vi "Lab09_task1.vi"() -> ()   [LabVIEW 2022 SP3]
uses:
  <vilib>/Utility/file.llb/Write Delimited Spreadsheet (string).vi
  <vilib>/Utility/file.llb/Write Delimited Spreadsheet (DBL).vi
  <vilib>/measure/mascope.llb/Pulse Measurements N chan.vi
  <vilib>/measure/NI_MAPro.lvlib
panel:
  out "Frequency (Hz)":dbl
  out "error out":errorcluster
  out "duty cycle":dbl[](array[numeric]) format="%.2p"
  out "pulse duration":dbl[](array[numeric]) format="%.2p"
  in  "reference levels":T1={"high ref level"=90.0, "mid ref level"=50.0, "low ref level"=10.0, "ref units"=1} {"ref units" items=["absolute", "percent"]; "high ref level" format="%.2p"; "low ref level" format="%.2p"; "mid ref level" format="%.2p"}
  out "period":dbl[](array[numeric]) format="%.2p"
  in  "file path (dialog if empty)":path
  in  "number of samples":i32=5000
  out "Waveform Graph":dynamicdata(graph)
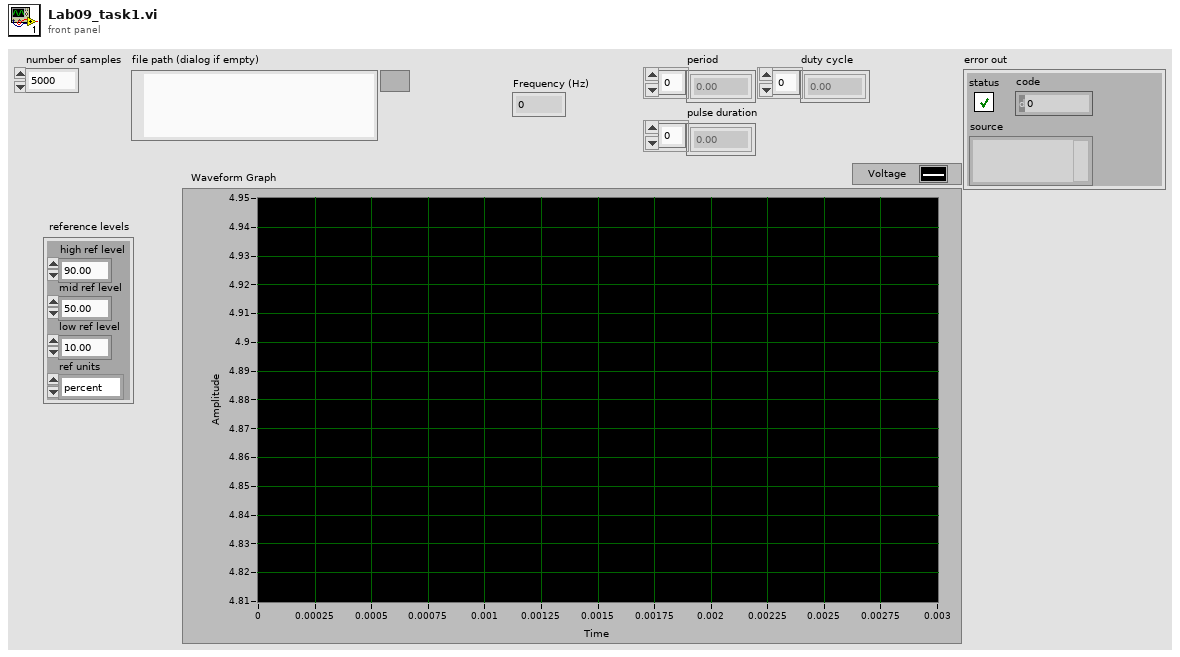
[diagram p1: front panel]
types:
  T1 = cluster{"high ref level":dbl, "mid ref level":dbl, "low ref level":dbl, "ref units":u16}
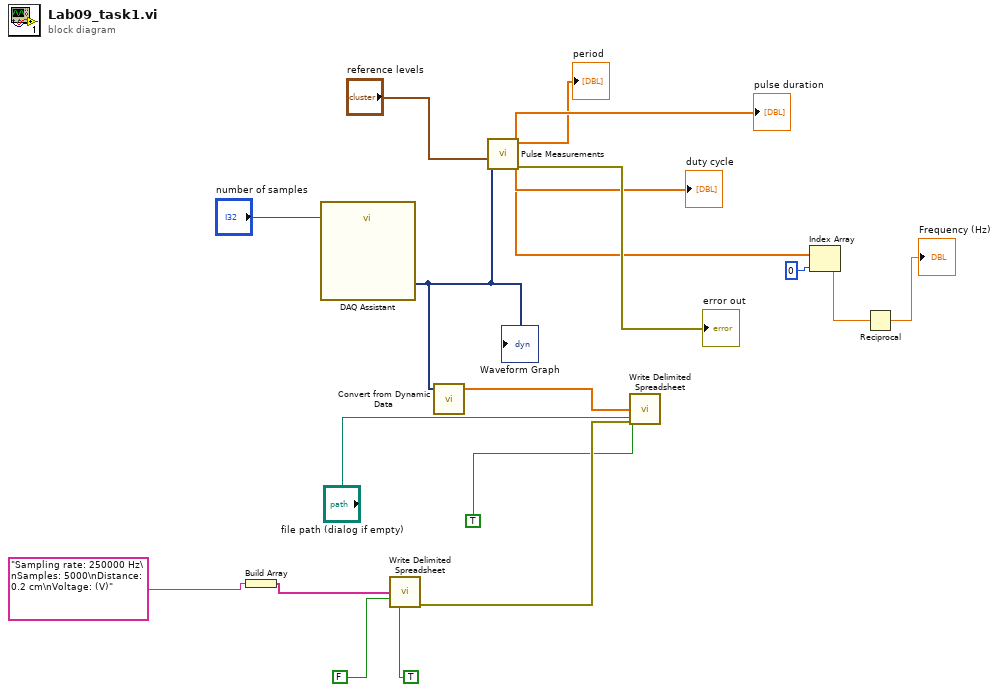
[diagram p0: block diagram]
diagram:
  n1 = Build Array("Sampling rate: 250000 Hz\nSamples: 5000\nDistance: 0.2 cm\nVoltage: (V)") -> (w16:string[])
  n2 = call "DAQ Assistant"("number of samples"="number of samples") -> ("data"=w9:dynamicdata)  [unwired: 16 in, 2 out]
  "Waveform Graph" <- w9
  n3 = call-poly <vilib>:"Write Delimited Spreadsheet.vi"("1D data"=w16, "append to file? (new file:F)"=FALSE, "transpose? (no:F)"=TRUE) -> ("error out"=w12:errorcluster)  [unwired: 11 in, 1 out]
  n4 = call "Convert from Dynamic Data"("Dynamic Data Type"=w9) -> ("Array"=w10:dbl[])  [unwired: 3 in]
  n5 = call-poly <vilib>:"Pulse Measurements.vi"("reference levels"="reference levels", "signal(s) in"=w9) -> ("error out"=→"error out":errorcluster, "duty cycle"=→"duty cycle":dbl[], "pulse duration"=→"pulse duration":dbl[], "period"=w1:dbl[])  [unwired: 5 in, 1 out]
  "period" <- w1
  n6 = call-poly <vilib>:"Write Delimited Spreadsheet.vi"("file path (dialog if empty)"="file path (dialog if empty)", "1D data"=w10, "append to file? (new file:F)"=TRUE, "error in (no error)"=w12) -> ()  [unwired: 10 in, 2 out]
  n7 = Index Array(array=w1, index=0) -> (element=w3:dbl)
  n8 = Reciprocal(x=w3) -> (1/x=→"Frequency (Hz)":dbl)
